vi "Get Register Address Limit.vi"(8 "error in (no error)":errorcluster, 11 "RFFE Command in":refnum<class "RFFE Command.lvclass">) -> (0 "error out":errorcluster, 2 "Register Address Limit":T1 format="%02x", 3 "RFFE Command out":refnum<class "RFFE Command.lvclass">)   [LabVIEW 2018, in "MIPI RFFE API.lvlib" / "RFFE Command.lvclass"]
uses:
  RFFE Command.lvclass
  Register Address.ctl
  MIPI RFFE API.lvlib
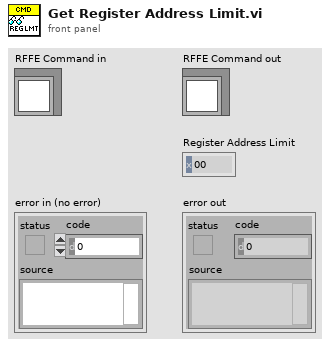
[diagram p1: front panel]
types:
  T1 = typedef "MIPI RFFE API.lvlib/Register Address.ctl" = u16
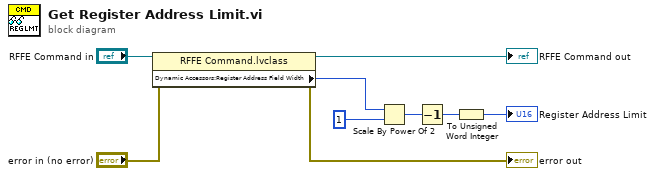
[diagram p0: block diagram]
diagram:
  n1 = property class="RFFE Command.lvclass"(reference="RFFE Command in", error in="error in (no error)") -> (reference out=→"RFFE Command out":refnum<class "RFFE Command.lvclass">, error out=→"error out":errorcluster, "Dynamic Accessors:Register Address Field Width"=w3:i32)
  n2 = Scale By Power Of 2(n=w3, x=1) -> (x*2^n=w2:i32)
  n3 = Decrement(x=w2) -> (x-1=w1:i32)
  n4 = To Unsigned Word Integer(number=w1) -> (unsigned 16bit integer=→"Register Address Limit":u16)
